vi "Odometry.vi"(10 "Radii (ft)":T1 {"Right Back Position" format="%.2f"; "Right Front Position" format="%.2f"; "Left Back Position" format="%.2f"; "Left Front Position" format="%.2f"}, 11 "(N-N-C-P) Swerve Motors":T2 {"Steer Scaling" format="%.2f"; "Drive Scaling" format="%.2f"; "Pod Locations (ft)"."Right Back Position" format="%.2f"; "Pod Locations (ft)"."Right Front Position" format="%.2f"; "Pod Locations (ft)"."Left Back Position" format="%.2f"; "Pod Locations (ft)"."Left Front Position" format="%.2f"}) -> ()   [LabVIEW 2023]
uses:
  <vilib>/Analysis/NI_AALPro.lvlib
  <vilib>/Analysis/coordinate.llb/2D Cartesian Coordinate Rotation (Scalar).vi
  <vilib>/Analysis/_algsub.llb/Real Vector Norm.vi
  Robot Global Data.vi
  <vilib>/ptbypt/NI_PtbyPt.lvlib
  swerve-template/Type Definitions/Data/Pod Positions.ctl
  <vilib>/REV Custom Controls/REVSparkRefnum.ctl
  <vilib>/REVLibDriver/REVLibDriver.lvlib
  swerve-template/Type Definitions/Hardware/Swerve Drives/(NEO-NEO-ThroughBore-Pigeon2) Swerve.ctl
panel:
  in  "Reset?":bool
  out "Robot Position (ft)":cluster{"x":dbl, "y":dbl, "theta":dbl}
  out "Robot Velocities (ft and deg)/s":cluster{"vx":dbl, "vy":dbl, "w":dbl}
  in  "Reset Pose":cluster{"vx":dbl, "vy":dbl, "w":dbl}
  out "Robot Pose":cluster{cluster{dbl, dbl}[]}[](graph)
  out "Speed":dbl
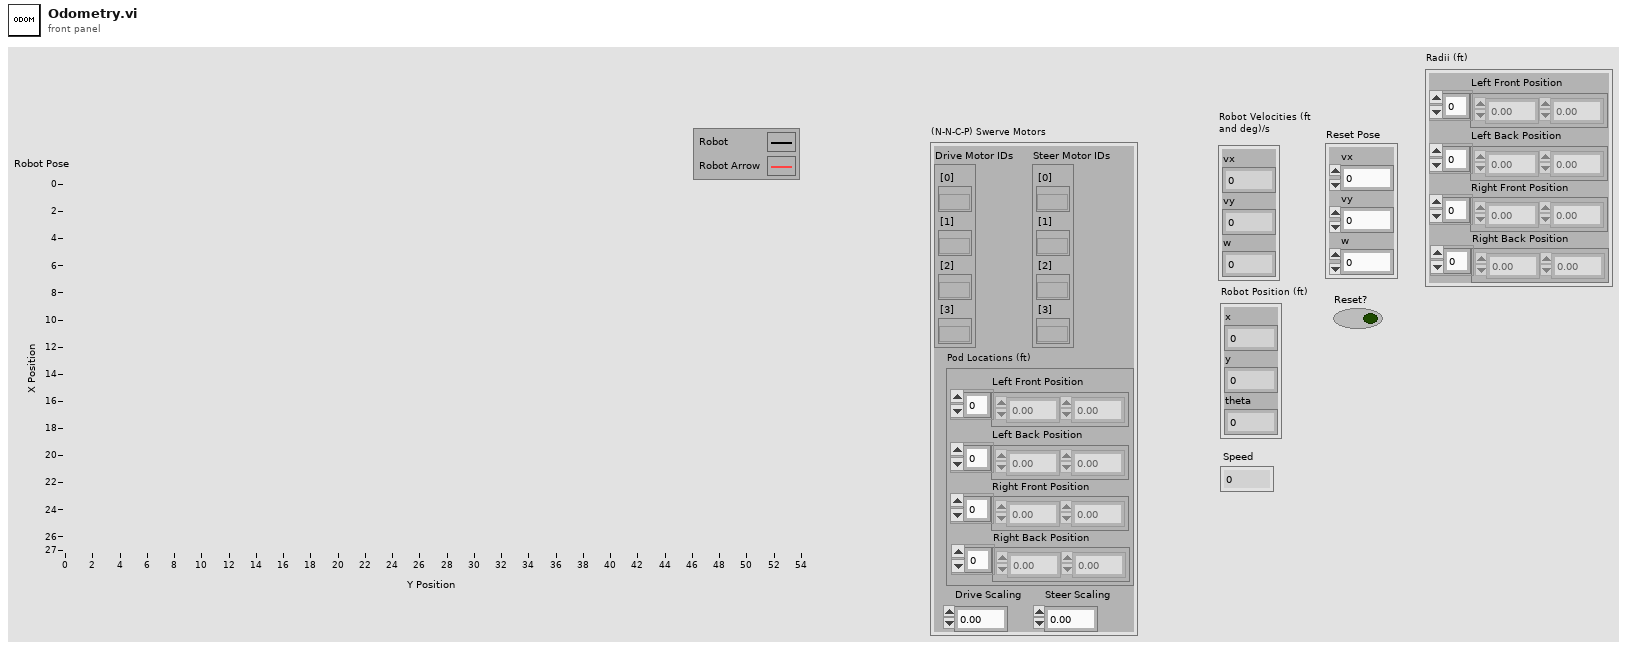
[diagram p1: front panel]
types:
  T1 = typedef "Pod Positions.ctl" = cluster{"Left Front Position":dbl[], "Left Back Position":dbl[], "Right Front Position":dbl[], "Right Back Position":dbl[]}
  T2 = typedef "(NEO-NEO-ThroughBore-Pigeon2) Swerve.ctl" = cluster{"Drive Motor IDs":cluster{"[0]":T3, "[1]":T3, "[2]":T3, "[3]":T3}, "Steer Motor IDs":cluster{"[0]":T3, "[1]":T3, "[2]":T3, "[3]":T3}, "Pod Locations (ft)":T1, "Drive Scaling":dbl, "Steer Scaling":dbl}
  T3 = typedef "REVLibDriver.lvlib/REVSparkRefnum.ctl" = refnum<k20>
  T4 = cluster{"Left Front":dbl, "Left Back":dbl, "Right Front":dbl, "Right Back":dbl}
  T5 = typedef "Robot Velocities.ctl" = cluster{"X Velocity":dbl, "Y Velocity":dbl, "Rotational \nVelocity":dbl}
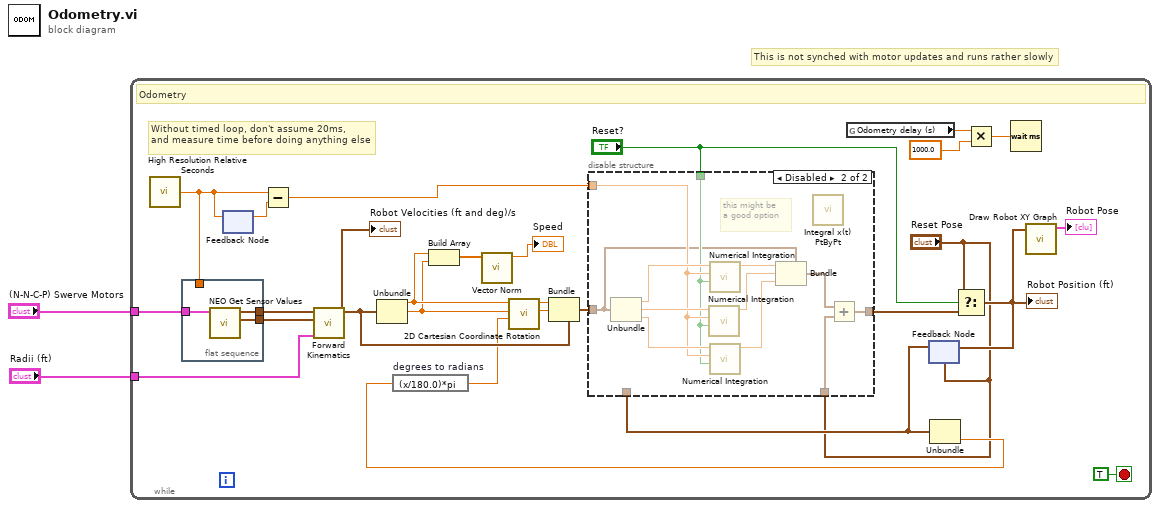
[diagram p0: block diagram]
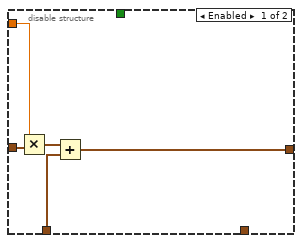
[diagram p2: hidden frame]
diagram:
  # "This is not synched with motor updates and runs rather slowly"
  n1 = while {
    tunnel: "(N-N-C-P) Swerve Motors" -> [w29]
    tunnel: "Radii (ft)" -> [w27]
    stop <- TRUE stop-if-true
    # "Without timed loop, don't assume 20ms,\nand measure time before doing anything else"
    # "Odometry"
    n2 = call <vilib>:"High Resolution Relative Seconds.vi"() -> ("relative seconds"=w6:dbl)
    n3 = flat-sequence {
      tunnel: w29 -> [w32]
      tunnel: [w31] -> w21
      tunnel: [w30] -> w20
      tunnel: w6 -> [_]
      frame #0 {
        n4 = call "NEO Get Sensor Values.vi"("Motors In"=w32) -> ("Steer Angles (degrees)"=w30:T4, "Drive Velocities (ft/s)"=w31:T4)  [unwired: 9 in]
      }
    }
    n5 = feedback-in #1(w6) -> ()
    n6 = feedback #1() -> (w8:dbl)  [unwired: 1 in]
    n7 = Subtract(x=w6, y=w8) -> (x-y=w7:dbl)
    n8 = call "Forward Kinematics.vi"("Radii (ft)"=w27, "Steer Angles (degrees)"=w20, "Drive Velocities (ft/s)"=w21) -> ("Robot Velocities (ft and deg)/s"=w25:T5)  [unwired: 8 in]
    "Robot Velocities (ft and deg)/s" <- w25
    n9 = Unbundle(w25) -> ("X Velocity"=w12:dbl, "Y Velocity"=w11:dbl)  [unwired: 1 out]
    n10 = Build Array(w12, w11) -> (w10:dbl[])
    n11 = call-poly <vilib>:"Vector Norm.vi"("Input Vector"=w10) -> ("norm"=→"Speed":dbl)  [unwired: 9 in, 1 out]
    n12 = global read "Robot Global Data.vi" "Odometry delay (s)"() -> (w5:dbl)
    n13 = feedback #2("Reset Pose") -> (w19:T5)
    n14 = Unbundle(w19) -> ("Rotational \nVelocity"=w15:dbl)  [unwired: 2 out]
    n15 = expression code="(x/180.0)*pi" "degrees to radians"(w15) -> (w18:dbl)
    n16 = call-poly <vilib>:"2D Cartesian Coordinate Rotation.vi"("theta"=w18, "y"=w11, "x"=w12) -> ("y out"=w23:dbl, "x out"=w24:dbl)  [unwired: 6 in, 1 out]
    n17 = Bundle(cluster=w25, "X Velocity"=w24, "Y Velocity"=w23) -> (w22:T5)  [unwired: 1 in]
    n18 = disable-structure shown="Disabled" {
      disable-tunnel: [w37 w39] -> w26
      disable-tunnel: w22 -> [w36 w43]
      disable-tunnel: w19 -> [w35 _]
      disable-tunnel: w7 -> [w34 w46]
      disable-tunnel: "Reset?" -> [_ w45]
      disable-tunnel: "Reset Pose" -> [_ w38]
      frame Enabled {
        n19 = Multiply(x=w34, y=w36) -> (x*y=w33:T5)
        n20 = Add(x=w33, y=w35) -> (x+y=w37:T5)
      }
      frame Disabled {
        # "this might be\na good option"
        n21 = Unbundle(w43) -> ("X Velocity"=w49:dbl, "Y Velocity"=w48:dbl, "Rotational \nVelocity"=w47:dbl)
        n22 = call "Numerical Integration.vi"("Reset?"=w45, "dt"=w46, "Data"=w48) -> ("Integrated Data"=w42:dbl)  [unwired: 8 in]
        n23 = call "Numerical Integration.vi"("Reset?"=w45, "dt"=w46, "Data"=w49) -> ("Integrated Data"=w44:dbl)  [unwired: 8 in]
        n24 = call "Numerical Integration.vi"("Reset?"=w45, "dt"=w46, "Data"=w47) -> ("Integrated Data"=w41:dbl)  [unwired: 8 in]
        n25 = Bundle(cluster=w43, "X Velocity"=w44, "Y Velocity"=w42, "Rotational \nVelocity"=w41) -> (w40:T5)
        n26 = call <vilib>:"Integral x(t) PtByPt.vi"() -> ()  [unwired: 4 in, 2 out]
        n27 = Add(x=w40, y=w38) -> (x+y=w39:T5)
      }
    }
    n28 = Select(t="Reset Pose", s="Reset?", f=w26) -> (s? t:f=w16:T5)
    "Robot Position (ft)" <- w16
    n29 = feedback-in #2(w16) -> ()
    n30 = Multiply(x=w5, y=1000.0) -> (x*y=w3:dbl)
    n31 = Wait (ms)(milliseconds to wait=w3) -> ()  [unwired: 1 out]
    n32 = call "Draw Robot XY Graph.vi"("Pose"=w16) -> ("Robot Pose"=→"Robot Pose":cluster{cluster{dbl, dbl}[]}[])  [unwired: 10 in]
  }
